vi "Set Path.vi"(8 "error in (no error)":errorcluster caption="에러 입력(에러 없음)", 9 "Filter path":T1, 10 "Input path":T2, 11 "CE RF Switch Box 입력":refnum<class "CE RF Switch Box.lvclass">) -> (0 "error out":errorcluster caption="에러 출력", 3 "CE RF Switch Box 출력":refnum<class "CE RF Switch Box.lvclass">)   [LabVIEW 2023, in "RF Switch Box.lvlib" / "CE RF Switch Box.lvclass"]
uses:
  CE RF Switch Box.lvclass
  CE RF Switch Box.lvclass/CE RF Switch Box.ctl
  Type Definition/Input path.ctl
  RF Switch Box.lvlib
  Type Definition/Filter path.ctl
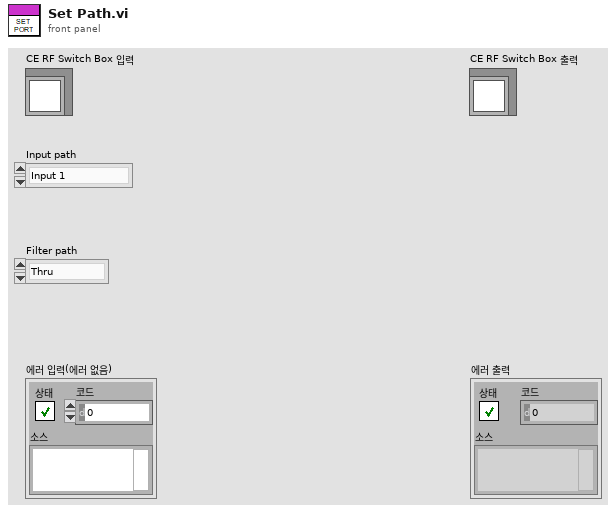
[diagram p1: front panel]
types:
  T1 = typedef "RF Switch Box.lvlib/Filter path.ctl" = enum16{"Thru", "Direct Amp", "1G HPF", "3G HPF", "7G HPF", "6G HPF", "port 1", "port 2", "port 3", "port 4", "port 5", "port 6", "port 7", "port 8", "port 9", "port 10", "port 11", "port 12", "port 13", "port 14", "port 15", "port 16", "port 17", "port 18"}
  T2 = typedef "RF Switch Box.lvlib/Input path.ctl" = enum16{"Input 1", "Input 2", "Input 3"}
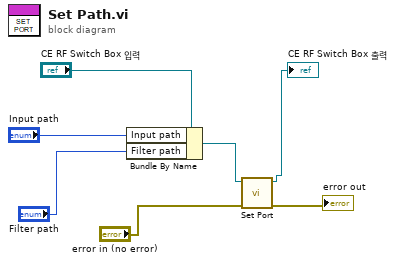
[diagram p0: block diagram]
diagram:
  n1 = Bundle By Name(cluster="CE RF Switch Box 입력", "Input path"="Input path", "Filter path"="Filter path") -> (w3:refnum<class "CE RF Switch Box.lvclass">)
  n2 = call "Set Port.vi"("error in (no error)"="error in (no error)", "CE RF Switch Box 입력"=w3) -> ("error out"=→"error out":errorcluster, "CE RF Switch Box 출력"=→"CE RF Switch Box 출력":refnum<class "CE RF Switch Box.lvclass">)  [unwired: 8 in]
